vi "Exmpl - Signal Generator.vi"() -> ()   [LabVIEW 2021]
doc: "::: CalcExpress Toolkit :::\nCopyright (c) 2000-2026 Konstantin Shifershteyn. All rights reserved."
uses:
  <vilib>/Utility/file.llb/Write To Spreadsheet File (DBL).vi
panel:
  out "Notification sent":string
  in  "phase":dbl[unit]=1.5707963267948966 format="%.1f"
  in  "GenReq":string="Generate"
  in  "stop":bool
  in  "noise amplitude":dbl=0.5 format="%.2f"
  in  "amplitude":dbl=1.0 format="%.2f"
  out "Signal":dbl[](graph)
  in  "cycles":i32=7
  in  "samples":i32=256
  in  "generate":bool
  in  "pass data through":T1(ring)
  in  "Notifier":string="COMM_Notifier"
  # "<<< click it to generate signal and send notification"
  # "<<< specifies a communication method to exchange data"
  # "Generation parameters"
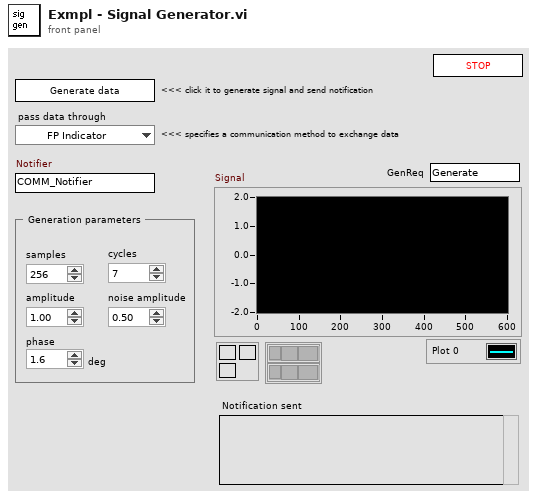
[diagram p1: front panel]
types:
  T1 = enum16{"FP Indicator", "File", "Queue", "VarMan variable"}
  T2 = enum32{"nothing", "reset", "assign name", "get name", "get handle"}
  T3 = enum16{"create", "destroy", "set value", "get value"}
  T4 = typedef "VarMan Variable Context Handle.ctl" = i32
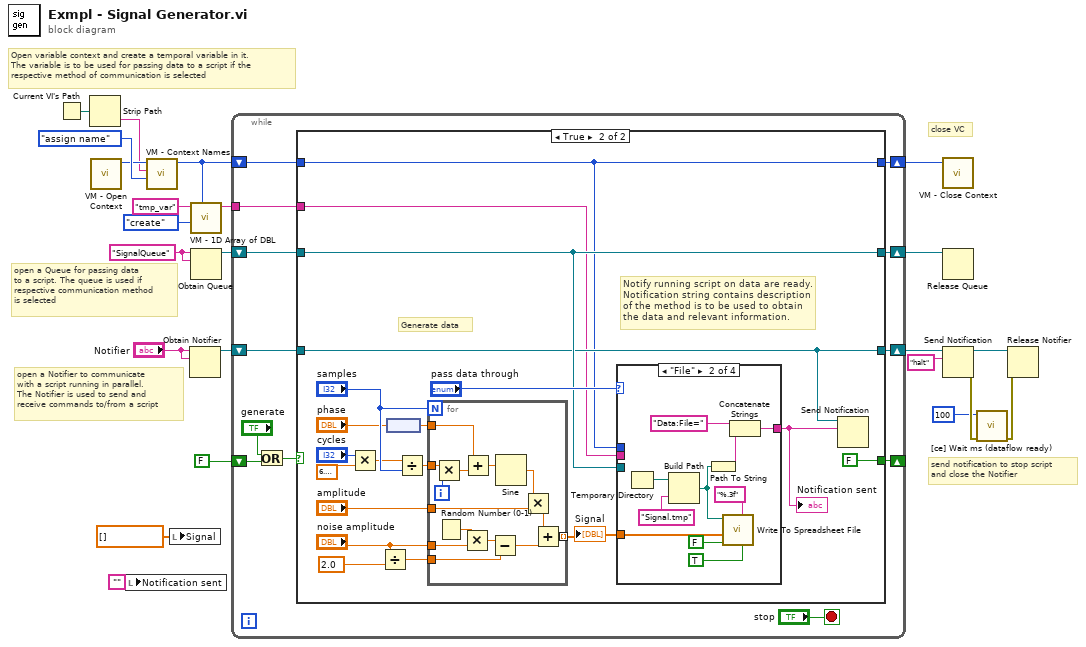
[diagram p0: block diagram]
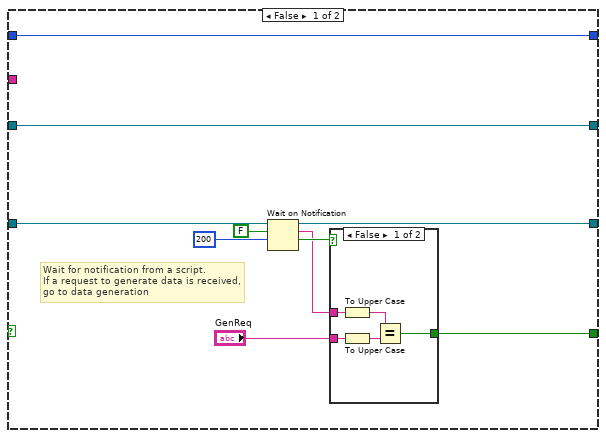
[diagram p2: hidden frame]
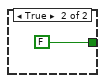
[diagram p3: hidden frame]
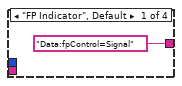
[diagram p4: hidden frame]
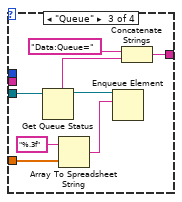
[diagram p5: hidden frame]
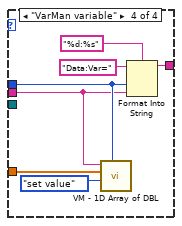
[diagram p6: hidden frame]
diagram:
  w4 = "SignalQueue"
  # "open a Queue for passing data\nto a script. The queue is used if\nrespective communication method\nis selected"
  # "close VC"
  # "Open variable context and create a temporal variable in it.\nThe variable is to be used for passing data to a script if the\nrespective method of communication is selected"
  # "open a Notifier to communicate\nwith a script running in parallel.\nThe Notifier is used to send and\nreceive commands to/from a script"
  # "send notification to stop script\nand close the Notifier"
  n1 = Current VI's Path() -> (path=w9:path)
  n2 = Strip Path(path=w9) -> (name=w10:string)  [unwired: 1 out]
  n3 = call "VM - Open Context.vi"() -> ("VC Handle out"=w11:T4)  [unwired: 9 in, 2 out]
  n4 = local write "Notification sent"("") -> ()
  n5 = call "VM - Context Names.vi"("action"=T2."assign name", "VC Name"=w10, "VC Handle"=w11) -> ("VC Handle out"=w2:T4)  [unwired: 3 in, 3 out]
  n6 = local write "Signal"(dbl[] [] ("Signal")) -> ()
  n7 = Obtain Notifier(name (unnamed)="Notifier", notification data type="Notifier") -> (notifier out=w23:refnum<notifier>)  [unwired: 2 in, 2 out]
  n8 = call "VM - 1D Array of DBL.vi"("VC Handle"=w2, "cmd"=T3."create", "name_spec"="tmp_var" ("name")) -> ("dup name_spec"=w16:string)  [unwired: 3 in, 5 out]
  n9 = Obtain Queue(name (unnamed)=w4, element data type=w4) -> (queue out=w22:refnum<queue>)  [unwired: 3 in, 2 out]
  n10 = while {
    tunnel: w16 -> [w25]
    shift-left: FALSE -> [w30]
    shift-right: [w31] -> _
    shift-right: [w33] -> w21
    shift-left: w22 -> [w34]
    shift-right: [w32] -> w15
    shift-left: w23 -> [w35]
    shift-right: [w26] -> w17
    shift-left: w2 -> [w27]
    stop <- "stop" stop-if-true
    n11 = Or(x="generate", y=w30) -> (x .or. y?=w28:bool)
    n12 = case shown="True" w28 {
      tunnel: w35 -> [w44 w63]
      tunnel: w34 -> [w45 w64]
      tunnel: [w45 w64] -> w33
      tunnel: [w43 w63] -> w32
      tunnel: [w37 FALSE] -> w31
      tunnel: w27 -> [w36 w56]
      tunnel: [w36 w56] -> w26
      tunnel: w25 -> [_ w57]
      frame False {
        # "Wait for notification from a script.\nIf a request to generate data is received,\ngo to data generation"
        n13 = Wait on Notification(notifier=w44, ignore previous (F)=FALSE ("ignore previous (T)"), timeout in ms (-1)=200 ("ms timeout (-1)")) -> (notifier out=w43:refnum<notifier>, notification=w39:string, timed out?=w40:bool)  [unwired: 1 in, 1 out]
        n14 = case shown="False" w40 {
          tunnel: w39 -> [w49 _]
          tunnel: "GenReq" -> [w50 _]
          tunnel: [w46 FALSE] -> w37
          frame False {
            n15 = To Upper Case(1:w49) -> (0:w48:string)
            n16 = To Upper Case(1:w50) -> (0:w47:string)
            n17 = Equal?(x=w48, y=w47) -> (x = y?=w46:bool)
          }
          frame True {
          }
        }
      }
      frame True {
        # "Notify running script on data are ready.\nNotification string contains description\nof the method is to be used to obtain\nthe data and relevant information."
        # "Generate data"
        n18 = Multiply(x="cycles", y=6.283185307179586) -> (x*y=w67:dbl)
        n19 = Divide(x="noise amplitude", y=2.0) -> (x/y=w59:dbl)
        n20 = node("phase") -> (w53:dbl)
        n21 = Divide(x=w67, y="samples") -> (x/y=w69:dbl)
        n22 = for {
          N: "samples" -> [_]
          tunnel: w69 -> [w100]
          tunnel: "amplitude" -> [w103]
          tunnel: [w110] -> w58 mode=indexing
          tunnel: "noise amplitude" -> [w107]
          tunnel: w59 -> [w105]
          tunnel: w53 -> [w97]
          i -> [w101]
          n23 = Multiply(x=w100, y=w101) -> (x*y=w99:dbl)
          n24 = Random Number (0-1)() -> (number: 0 to 1=w108:dbl)
          n25 = Multiply(x=w108, y=w107) -> (x*y=w106:dbl)
          n26 = Add(x=w97, y=w99) -> (x+y=w98:dbl)
          n27 = Subtract(x=w106, y=w105) -> (x-y=w104:dbl)
          n28 = Sine(x=w98) -> (sin(x)=w102:dbl)
          n29 = Multiply(x=w102, y=w103) -> (x*y=w109:dbl)
          n30 = Add(x=w109, y=w104) -> (x+y=w110:dbl)
        }
        "Signal" <- w58
        n31 = case shown="\"File\"" "pass data through" {
          tunnel: ["Data:fpControl=Signal" w80 w88 w90] -> w52
          tunnel: w58 -> [_ w77 w87 w96]
          tunnel: w64 -> [_ _ w84 _]
          tunnel: w57 -> [_ _ _ w91]
          tunnel: w56 -> [_ _ _ w92]
          frame "FP Indicator", Default {
          }
          frame "File" {
            n32 = Temporary Directory() -> (w79:path)
            n33 = Build Path(base path=w79, name or relative path="Signal.tmp") -> (appended path=w73:path)
            n34 = Path To String(path=w73) -> (string=w72:string)
            n35 = call-poly <vilib>:"Write To Spreadsheet File.vi"("transpose? (no:F)"=TRUE, "format (%.3f)"="%.3f", "append to file? (new file:F)"=FALSE, "1D data"=w77, "file path (dialog if empty)"=w73) -> ()  [unwired: 3 in, 1 out]
            n36 = Concatenate Strings("Data:File=", w72) -> (w80:string)
          }
          frame "Queue" {
            n37 = Get Queue Status(queue=w84) -> (queue out=w83:refnum<queue>, queue name=w82:string)  [unwired: 2 in, 6 out]
            n38 = Array To Spreadsheet String(array=w87, 3:"%.3f" ("format string")) -> (spreadsheet string=w86:string)  [unwired: 1 in]
            n39 = Enqueue Element(queue=w83, element=w86) -> ()  [unwired: 2 in, 3 out]
            n40 = Concatenate Strings("Data:Queue=", w82) -> (w88:string)
          }
          frame "VarMan variable" {
            n41 = call "VM - 1D Array of DBL.vi"("VC Handle"=w92, "cmd"=T3."set value", "value in"=w96, "name_spec"=w91) -> ()  [unwired: 2 in, 6 out]
            n42 = Format Into String(format string="%d:%s", initial string="Data:Var=", w92, w91) -> (resulting string=w90:string)  [unwired: 1 in, 1 out]
          }
        }
        "Notification sent" <- w52
        n43 = Send Notification(notification=w52, notifier=w63) -> ()  [unwired: 1 in, 2 out]
      }
    }
  }
  n44 = call "VM - Close Context.vi"("VC Handle"=w17) -> ()  [unwired: 9 in, 2 out]
  n45 = Release Queue(queue=w21) -> ()  [unwired: 2 in, 3 out]
  n46 = Send Notification(notification="halt", notifier=w15) -> (notifier out=w14:refnum<notifier>, error out=w8:errorcluster)  [unwired: 1 in]
  n47 = call "[ce] Wait ms (dataflow ready).vi"("error in"=w8, "milliseconds to wait"=u32 100) -> ("error out"=w7:errorcluster)  [unwired: 3 in, 4 out]
  n48 = Release Notifier(notifier=w14, error in (no error)=w7) -> ()  [unwired: 1 in, 3 out]
